vi "Tree_HierarchicalPath_Tests.vi"(11 "error in":errorcluster) -> (15 "error out":errorcluster)   [LabVIEW 2016, in "DronaTest.lvlib"]
uses:
  DronaTest.lvlib
  APIs/Stimulus/ControlValue/SetValueAuto.vi
  APIs/Stimulus/ControlValue/Controls/Tree/SetValueByHierarchicalPath.vi
  APIs/Assert/AssertControlValue/Equal.vi
  APIs/Get/GetControlRef/GetControlRefByPath.vi
  <vilib>/addons/_JKI Toolkits/Caraya/classes/Test/Test.lvclass
  Drona.lvlib
  <vilib>/SLL Toolkit/SLL Debug/SLL Debug.lvlib
  APIs/Assert/AssertControlValue/AssertControlValue.lvlib
  APIs/Stimulus/ControlValue/ControlValue.lvlib
  <vilib>/addons/_JKI Toolkits/Caraya/classes/Assert/Assert.lvclass
  APIs/Stimulus/ControlValue/Controls/Tree/StimulusTree.lvlib
  APIs/Get/GetControlRef/GetControlRef.lvlib
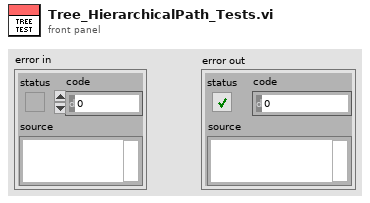
[diagram p1: front panel]
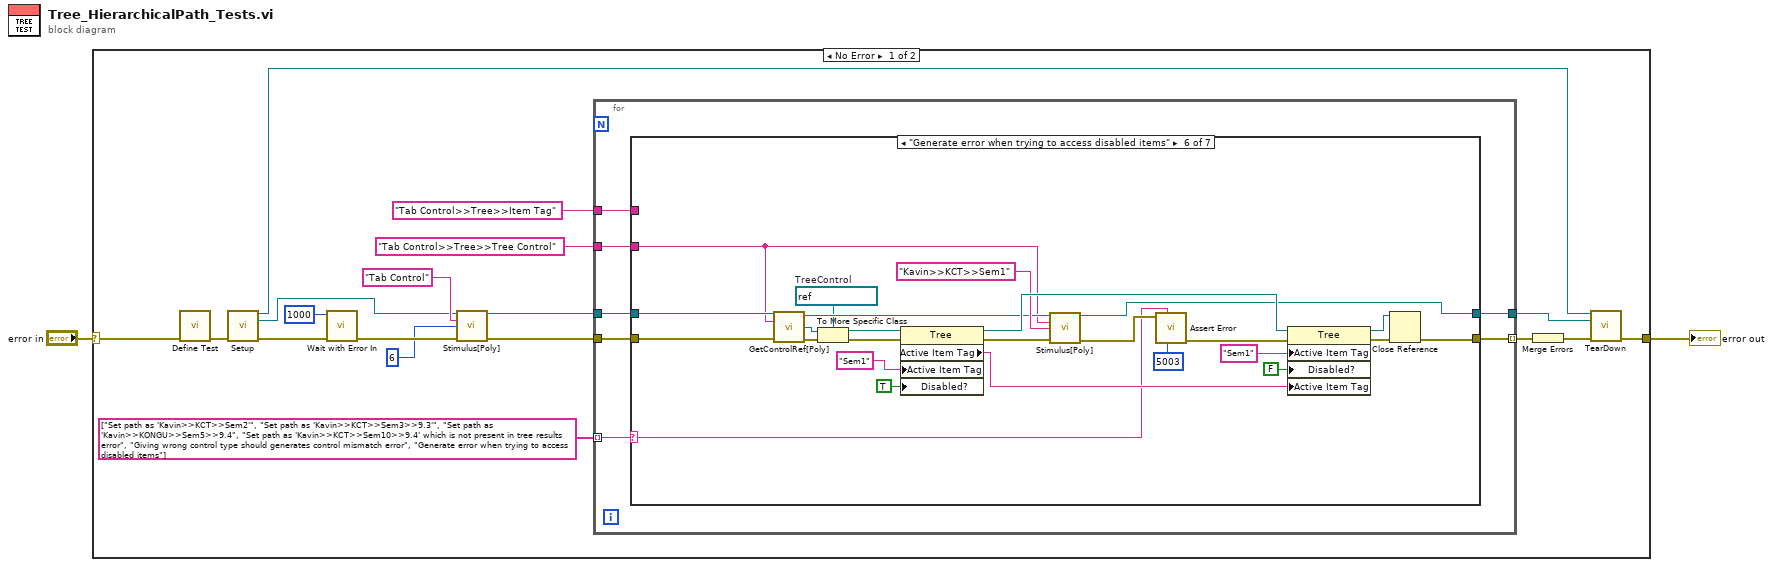
[diagram p0: block diagram]
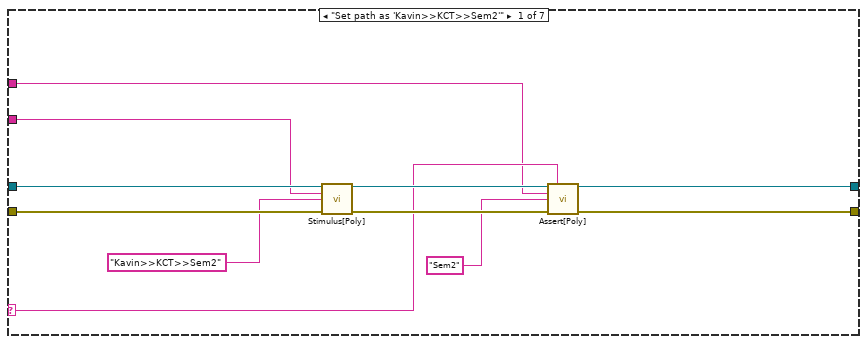
[diagram p2: hidden frame]
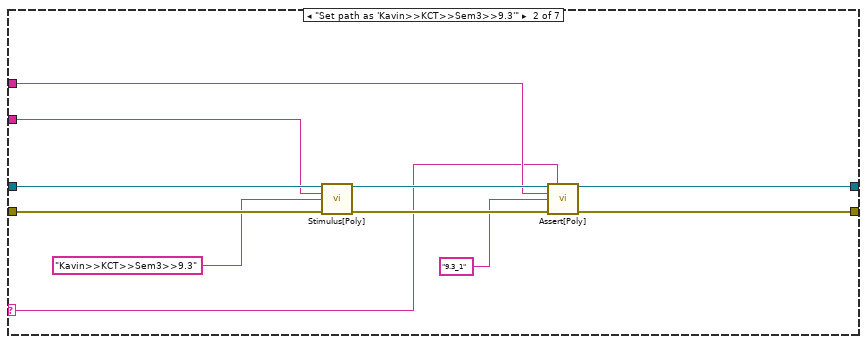
[diagram p3: hidden frame]
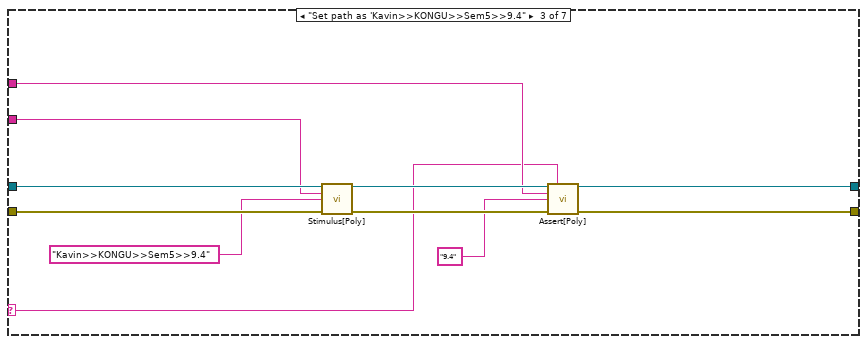
[diagram p4: hidden frame]
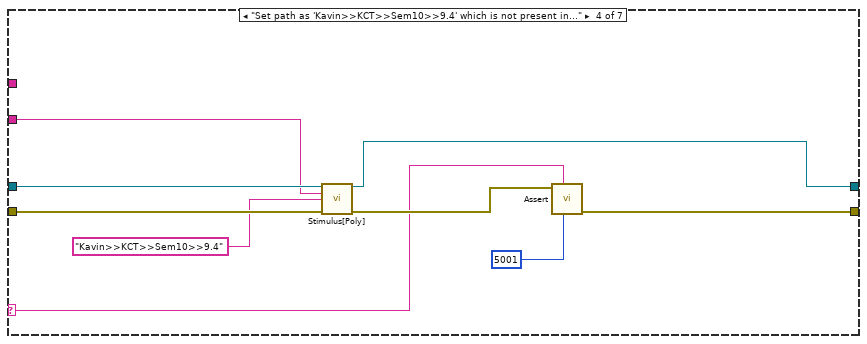
[diagram p5: hidden frame]
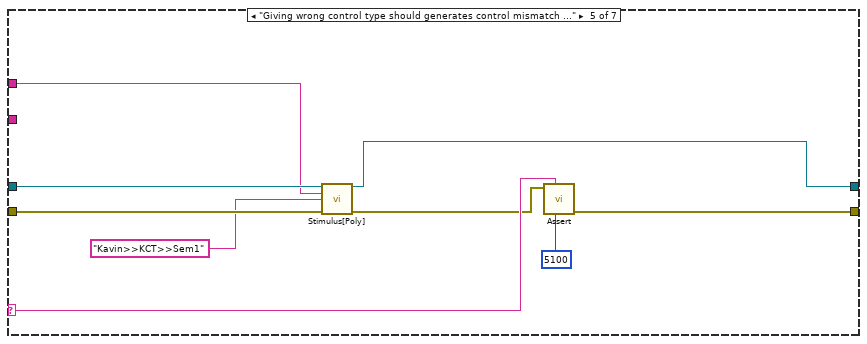
[diagram p6: hidden frame]
diagram:
  n1 = case shown="No Error" "error in" {
    selector: "error in" -> [w20 w106]
    tunnel: [w3 w106] -> w1
    frame No Error {
      n2 = call <vilib>:"Define Test.vi"("error in (no error)"=w20) -> ("error out"=w9:errorcluster)  [unwired: 9 in, 1 out]
      n3 = call "Setup.vi"("error in"=w9) -> ("Application Ref"=w4:refnum<vi>, "VI out"=w8:refnum<vi>, "error out"=w7:errorcluster)  [unwired: 12 in]
      n4 = call <vilib>:"Wait with Error In.vi"("error in (no error)"=w7, "milliseconds to wait"=u32 1000) -> ("error out"=w18:errorcluster)  [unwired: 9 in]
      n5 = call-poly "Stimulus[Poly].vi"("VI Reference In"=w8, "Control Path"="Tab Control", "Value (Signaling)"=6, "error in"=w18) -> ("VI Reference Out"=w14:refnum<vi>, "error out"=w17:errorcluster)  [unwired: 10 in]
      n6 = for {
        tunnel: w14 -> [w26]
        tunnel: "Tab Control>>Tree>>Tree Control" ("Control Path") -> [w25]
        tunnel: "Tab Control>>Tree>>Item Tag" ("Control Path") -> [w24]
        tunnel: string[] ["Set path as 'Kavin>>KCT>>Sem2'", "Set path as 'Kavin>>KCT>>Sem3>>9.3'", "Set path as 'Kavin>>KONGU>>Sem5>>9.4", "Set path as 'Kavin>>KCT>>Sem10>>9.4' which is not present in tree results error", "Giving wrong control type should generates control mismatch error", "Generate error when trying to access disabled items"] -> [w22] mode=indexing
        tunnel: [w21] -> w5
        tunnel: w17 -> [w27]
        tunnel: [w23] -> w10 mode=indexing
        n7 = case shown="\"Generate error when trying to access disabled items\"" w22 {
          selector: w22 -> [w32 w41 w52 w62 w75 w82 _]
          tunnel: w27 -> [w38 w49 w60 w69 w78 w83 w105]
          tunnel: w26 -> [w37 w48 w59 w68 w77 w84 w104]
          tunnel: w25 -> [w30 w45 w56 w67 _ w79 _]
          tunnel: w24 -> [w31 w44 w55 _ w70 _ _]
          tunnel: [w34 w43 w54 w66 w76 w80 w105] -> w23
          tunnel: [w33 w42 w53 w65 w74 w81 w104] -> w21
          frame "Set path as 'Kavin>>KCT>>Sem2'" {
            n8 = call-poly "Stimulus[Poly].vi"("VI Reference In"=w37, "Control Path"=w30, "Hierarchical Path"="Kavin>>KCT>>Sem2" ("Item Name"), "Error In"=w38) -> ("VI Reference Out"=w35:refnum<vi>, "Error Out"=w36:errorcluster)  [unwired: 10 in]
            n9 = call-poly "Assert[Poly].vi"("VI Reference In"=w35, "Test Label"=w32, "Control Path"=w31, "Control Value"="Sem2", "Error In"=w36) -> ("VI Reference Out"=w33:refnum<vi>, "Error Out"=w34:errorcluster)  [unwired: 8 in, 1 out]
          }
          frame "Set path as 'Kavin>>KCT>>Sem3>>9.3'" {
            n10 = call-poly "Stimulus[Poly].vi"("VI Reference In"=w48, "Control Path"=w45, "Hierarchical Path"="Kavin>>KCT>>Sem3>>9.3" ("Item Name"), "Error In"=w49) -> ("VI Reference Out"=w46:refnum<vi>, "Error Out"=w47:errorcluster)  [unwired: 10 in]
            n11 = call-poly "Assert[Poly].vi"("VI Reference In"=w46, "Test Label"=w41, "Control Path"=w44, "Control Value"="9.3_1", "Error In"=w47) -> ("VI Reference Out"=w42:refnum<vi>, "Error Out"=w43:errorcluster)  [unwired: 8 in, 1 out]
          }
          frame "Set path as 'Kavin>>KONGU>>Sem5>>9.4" {
            n12 = call-poly "Stimulus[Poly].vi"("VI Reference In"=w59, "Control Path"=w56, "Hierarchical Path"="Kavin>>KONGU>>Sem5>>9.4" ("Item Name"), "Error In"=w60) -> ("VI Reference Out"=w57:refnum<vi>, "Error Out"=w58:errorcluster)  [unwired: 10 in]
            n13 = call-poly "Assert[Poly].vi"("VI Reference In"=w57, "Test Label"=w52, "Control Path"=w55, "Control Value"="9.4" ("Item Name"), "Error In"=w58) -> ("VI Reference Out"=w53:refnum<vi>, "Error Out"=w54:errorcluster)  [unwired: 8 in, 1 out]
          }
          frame "Set path as 'Kavin>>KCT>>Sem10>>9.4' which is not present in tree results error" {
            n14 = call-poly "Stimulus[Poly].vi"("VI Reference In"=w68, "Control Path"=w67, "Hierarchical Path"="Kavin>>KCT>>Sem10>>9.4" ("Item Name"), "Error In"=w69) -> ("VI Reference Out"=w65:refnum<vi>, "Error Out"=w63:errorcluster)  [unwired: 10 in]
            n15 = call-poly <vilib>:"Assert.vi"("error code (1)"=5001, "Label"=w62, "Error?"=w63) -> ("error out"=w66:errorcluster)  [unwired: 7 in, 1 out]
          }
          frame "Giving wrong control type should generates control mismatch error" {
            n16 = call-poly "Stimulus[Poly].vi"("VI Reference In"=w77, "Control Path"=w70, "Hierarchical Path"="Kavin>>KCT>>Sem1" ("Item Name"), "Error In"=w78) -> ("VI Reference Out"=w74:refnum<vi>, "Error Out"=w72:errorcluster)  [unwired: 10 in]
            n17 = call-poly <vilib>:"Assert.vi"("error code (1)"=5100, "Label"=w75, "Error?"=w72) -> ("error out"=w76:errorcluster)  [unwired: 7 in, 1 out]
          }
          frame "Generate error when trying to access disabled items" {
            w88 = refnum<vi> refnum  # TreeControl
            n18 = call-poly "GetControlRef[Poly].vi"("VI Reference In"=w84, "Control Path"=w79, "error In"=w83) -> ("VI Reference Out"=w95:refnum<vi>, "Ctl Refnum"=w87:refnum<vi>, "error out"=w85:errorcluster)  [unwired: 10 in]
            n19 = To More Specific Class(target class=w88, reference=w87, error in=w85) -> (specific class reference=w89:refnum<vi>, error out=w86:errorcluster)
            n20 = property class="Tree"(reference=w89, error in=w86, "Active Item Tag"="Sem1" ("Active Item:Tag"), "Disabled?"=TRUE ("Active Item:Disabled?")) -> (reference out=w100:refnum<vi>, error out=w94:errorcluster, "Active Item Tag"=w101:string)
            n21 = call-poly "Stimulus[Poly].vi"("VI Reference In"=w95, "Control Path"=w79, "Hierarchical Path"="Kavin>>KCT>>Sem1" ("Item Tag"), "Error In"=w94) -> ("VI Reference Out"=w81:refnum<vi>, "Error Out"=w97:errorcluster)  [unwired: 10 in]
            n22 = call <vilib>:"Assert Error.vi"("error code (1)"=5003, "Label"=w82, "Error?"=w97) -> ("error out"=w98:errorcluster)  [unwired: 7 in, 1 out]
            n23 = property class="Tree"(reference=w100, error in=w98, "Active Item Tag"="Sem1" ("Active Item:Tag"), "Disabled?"=FALSE ("Active Item:Disabled?"), "Active Item Tag"=w101) -> (reference out=w93:refnum<vi>, error out=w92:errorcluster)
            n24 = Close Reference(reference=w93, error in (no error)=w92) -> (error out=w80:errorcluster)
          }
          frame Default {
          }
        }
      }
      n25 = Merge Errors(w10) -> (w6:errorcluster)
      n26 = call "TearDown.vi"("Application Ref"=w4, "VI in"=w5, "error in (no error)"=w6) -> ("error out"=w3:errorcluster)  [unwired: 12 in]
    }
    frame Error {
    }
  }
  "error out" <- w1
